vi "Write App INI.vi"(6 "Node":string, 8 "error in (no error)":errorcluster, 9 "Cluster":string, 10 "System":string, 11 "System Config Module in":refnum<class "System Config Module.lvclass">) -> (0 "error out":errorcluster, 2 "Main Config Path":path, 3 "System Config Module out":refnum<class "System Config Module.lvclass">, 4 "INI Path":path)   [LabVIEW 2020, in "Volatus.lvlib" / "System Config Module.lvclass"]
uses:
  System Config Module.lvclass
  System Config Module.lvclass/System Config Module.ctl
  <vilib>/Utility/config.llb/Write Key (String).vi
  <vilib>/Utility/config.llb/Read Key (String).vi
  Volatus.lvlib
  <vilib>/Utility/config.llb/NI_LVConfig.lvlib
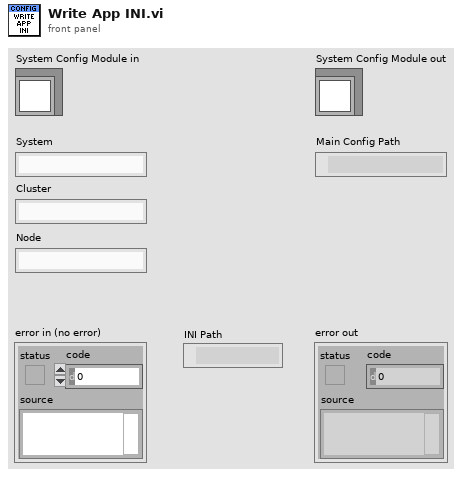
[diagram p1: front panel]
types:
  T1 = typedef "NI_LVConfig.lvlib/Config Data RefNum.ctl" = refnum<k1>
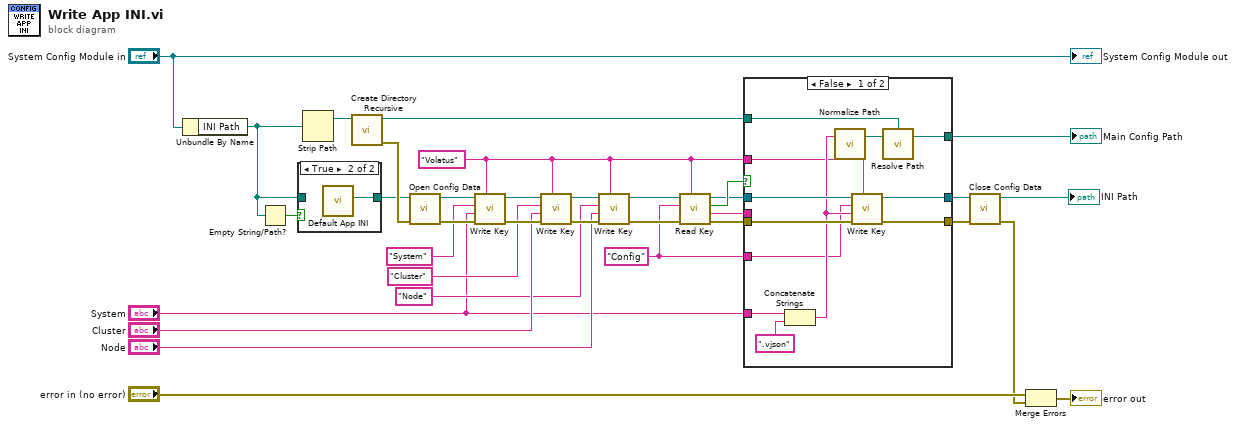
[diagram p0: block diagram]
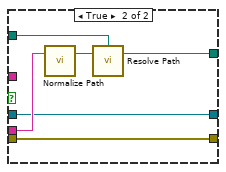
[diagram p3: hidden frame]
diagram:
  w8 = "Config"
  w14 = "Volatus" ("section")
  n1 = Unbundle By Name("System Config Module in") -> ("INI Path"=w11:path)
  n2 = Empty String/Path?(string/path=w11) -> (empty?=w31:bool)
  n3 = case shown="True" w31 {
    tunnel: w11 -> [w35 _]
    tunnel: [w35 w36] -> w30
    frame False {
    }
    frame True {
      n4 = call "Default App INI.vi"() -> ("Default App INI"=w36:path)  [unwired: 11 in]
    }
  }
  n5 = Strip Path(path=w11) -> (stripped path=w2:path)  [unwired: 1 out]
  n6 = call <vilib>:"Create Directory Recursive.vi"("directory"=w2) -> ("error out"=w34:errorcluster, "directory copy"=w1:path)  [unwired: 4 in, 1 out]
  n7 = call <vilib>:"Open Config Data.vi"("error in (no error)"=w34, "configuration file path"=w30) -> ("error out"=w22:errorcluster, "refnum"=w29:T1)  [unwired: 7 in, 1 out]
  n8 = call-poly <vilib>:"Write Key.vi"("section"=w14, "error in (no error)"=w22, "value"="System", "key"="System", "refnum"=w29) -> ("error out"=w23:errorcluster, "refnum out"=w28:T1)  [unwired: 4 in, 1 out]
  n9 = call-poly <vilib>:"Write Key.vi"("section"=w14, "error in (no error)"=w23, "value"="Cluster", "key"="Cluster", "refnum"=w28) -> ("error out"=w24:errorcluster, "refnum out"=w27:T1)  [unwired: 4 in, 1 out]
  n10 = call-poly <vilib>:"Write Key.vi"("section"=w14, "error in (no error)"=w24, "value"="Node", "key"="Node", "refnum"=w27) -> ("error out"=w25:errorcluster, "refnum out"=w26:T1)  [unwired: 4 in, 1 out]
  n11 = call-poly <vilib>:"Read Key.vi"("section"=w14, "error in (no error)"=w25, "key"=w8, "refnum"=w26) -> ("error out"=w13:errorcluster, "value"=w12:string, "found?"=w16:bool, "refnum out"=w15:T1)  [unwired: 4 in]
  n12 = case shown="False" w16 {
    tunnel: w15 -> [w43 w50]
    tunnel: w14 -> [w40 _]
    tunnel: w13 -> [w42 w49]
    tunnel: w12 -> [_ w53]
    tunnel: w1 -> [w45 w52]
    tunnel: [w44 w51] -> w10
    tunnel: "System" -> [w47 _]
    tunnel: w8 -> [w39 _]
    tunnel: [w38 w50] -> w7
    tunnel: [w37 w49] -> w6
    frame False {
      n13 = Concatenate Strings(w47, ".vjson" ("string")) -> (w41:string)
      n14 = call "Normalize Path.vi"("Path String"=w41) -> ("Path"=w48:path)  [unwired: 2 in]
      n15 = call-poly <vilib>:"Write Key.vi"("section"=w40, "error in (no error)"=w42, "value"=w41, "key"=w39, "refnum"=w43) -> ("error out"=w37:errorcluster, "refnum out"=w38:T1)  [unwired: 4 in, 1 out]
      n16 = call "Resolve Path.vi"("Starting Path"=w45, "Path"=w48) -> ("Resolved Path"=w44:path)  [unwired: 4 in]
    }
    frame True {
      n17 = call "Normalize Path.vi"("Path String"=w53) -> ("Path"=w54:path)  [unwired: 2 in]
      n18 = call "Resolve Path.vi"("Starting Path"=w52, "Path"=w54) -> ("Resolved Path"=w51:path)  [unwired: 4 in]
    }
  }
  "Main Config Path" <- w10
  n19 = call <vilib>:"Close Config Data.vi"("error in (no error)"=w6, "refnum"=w7) -> ("error out"=w4:errorcluster, "file path"=→"INI Path":path)  [unwired: 8 in]
  n20 = Merge Errors("error in (no error)", w4) -> (→"error out":errorcluster)
  "System Config Module out" <- "System Config Module in"
